vi "Parse Load SA Precision Setting.vi"(8 "error in (no error)":errorcluster caption="에러 입력(에러 없음)", 10 "JSON string":string, 11 "Instrument Manager 입력":refnum<class "Instrument Manager.lvclass">) -> (0 "error out":errorcluster caption="에러 출력", 1 "Params":cluster{"Peak Frequency":dbl, "Sweep Time":dbl}, 2 "Load SA Precision Setting Param":T1, 3 "Instrument Manager 출력":refnum<class "Instrument Manager.lvclass">)   [LabVIEW 2023, in "Instrument Manager.lvclass"]
uses:
  Instrument Manager.lvclass
  Param Definition/Load SA Precision Setting Param.ctl
  Instrument Manager.lvclass/Instrument Manager.ctl
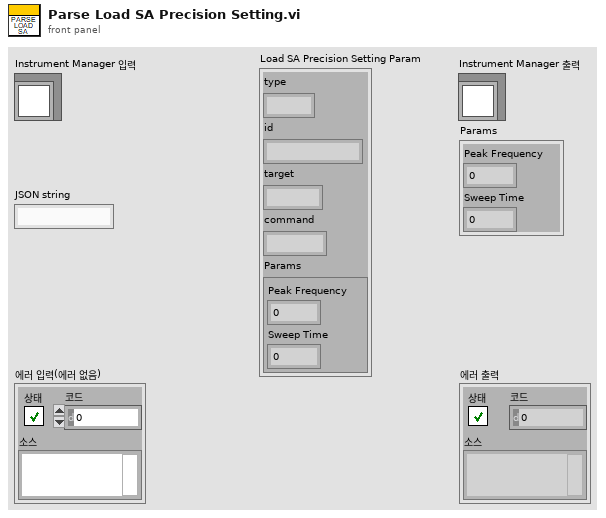
[diagram p1: front panel]
types:
  T1 = typedef "Instrument Manager.lvclass/Load SA Precision Setting Param.ctl" = cluster{"type":string, "id":string, "target":string, "command":string, "Params":cluster{"Peak Frequency":dbl, "Sweep Time":dbl}}
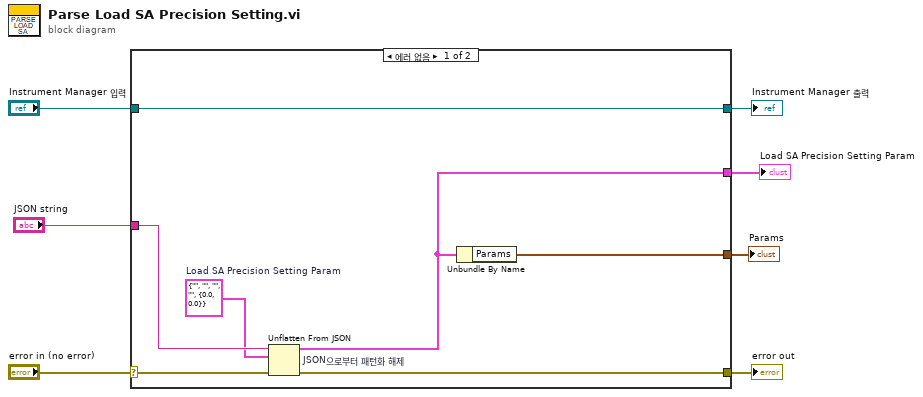
[diagram p0: block diagram]
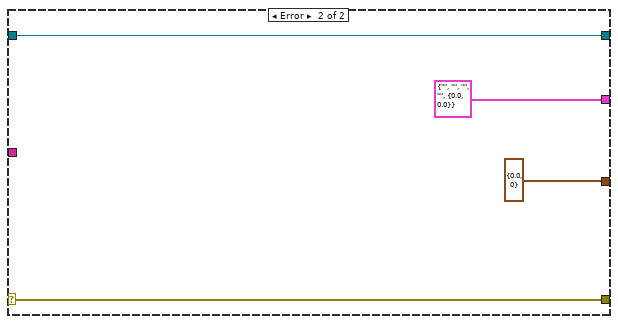
[diagram p2: hidden frame]
diagram:
  n1 = case shown="에러 없음" "error in (no error)" {
    selector: "error in (no error)" -> [w13 w18]
    tunnel: [w10 w18] -> w6
    tunnel: [w14 w17] -> w4
    tunnel: "Instrument Manager 입력" -> [w14 w17]
    tunnel: "JSON string" -> [w12 _]
    tunnel: [w9 T1 {"type"="", "id"="", "target"="", "command"="", "Params"={"Peak Frequency"=0.0, "Sweep Time"=0.0}} ("Load SA Precision Setting Param")] -> w2
    tunnel: [w8 cluster{"Peak Frequency":dbl, "Sweep Time":i32} {"Peak Frequency"=0.0, "Sweep Time"=0} ("Params")] -> w1
    frame No Error {
      w11 = T1 {"type"="", "id"="", "target"="", "command"="", "Params"={"Peak Frequency"=0.0, "Sweep Time"=0.0}}  # Load SA Precision Setting Param
      n2 = Unflatten From JSON "JSON으로부터 패턴화 해제"(JSON string=w12, type and defaults=w11, error in (no error)=w13) -> (value=w9:T1, error out=w10:errorcluster)  [unwired: 4 in]
      n3 = Unbundle By Name(w9) -> ("Params"=w8:cluster{"Peak Frequency":dbl, "Sweep Time":dbl})
    }
    frame Error {
    }
  }
  "error out" <- w6
  "Instrument Manager 출력" <- w4
  "Load SA Precision Setting Param" <- w2
  "Params" <- w1
